vi "waveform-frontpanel.vi"() -> ()   [LabVIEW 2026]
doc: "波形图界面 - 测控软件 多链路实时波形展示。仅前面板布局演示，无程序逻辑。来源：波形图.html 主界面。"
panel:
  out "运行时长":string="运行时长: 00:00:00"
  out "通道":string="通道: 16"
  out "视图":string="视图: 0.0 - 30.0 s"
  out "窗口":string="窗口: 30.0 s"
  out "采样率":string="采样率: 100 Hz / 10 Hz"
  out "链路":string="链路: 4/4 在线"
  out "?":string="滚轮:缩放时间轴 · 左键框选放大 · 右键平移 · 双击复位"
  out "?":string="Δ值 --"
  out "?":string="Δt --"
  out "?":string="C2 --"
  out "?":string="C1 --"
  out "?":string="测量游标未放置 (0/2)"
  out "?":bool
  out "ARINC429 链路":bool=TRUE
  out "CAN 链路":bool=TRUE
  out "OPC 链路":bool=TRUE
  out "TCP 链路":bool=TRUE
  out "可见通道":i32=16
  out "总通道数":i32=23
  out "绘制帧率":string="60 fps"
  out "重绘周期":string="50 ms"
  out "?":string[](array[string])=["\n● 下位机 TCP（100 Hz · 10 通道）\n  ■ 转速 (rpm)\n  ■ 扭矩 (N·m)\n  ■ 排气温度 (℃)\n  ■ 滑油压力 (kPa)\n  ■ 燃油流量 (kg/h)\n  ■ 振动 (g)\n  ■ 进气温度 (℃)\n  ■ 滑油温度 (℃)\n  ■ 启动信号\n  ■ 点火状态\n\n────────────────────────────────\n\n● PLC OPC（10 Hz · 5 通道）\n  ■ 28V 母线电压 (V)\n  ■ 28V 母线电流 (A)\n  ■ 环境温度 (℃)\n  ■ 气源压力 (kPa)\n  ■ 气动阀状态\n\n────────────────────────────────\n\n● CAN 总线（50 Hz · 4 通道）\n  ■ 发电机频率 (Hz)\n  ■ 母线电压 (V)\n  ■ 母线电流 (A)\n  ■ 发电机状态\n\n\n"]
  out "?":waveform(dbl)(graph)
  out "?":string[](array[string])=["\n● 下位机 TCP  ·  在线\n  192.168.1.101:8000\n  PXIC-8840 环形缓冲 · 采样 100 Hz\n  通道 10 个\n\n\n\n\n──────────────────────────────\n\n\n\n\n● PLC OPC  ·  在线\n  opc.tcp://192.168.1.50:4840\n  西门子 S7-1500 · OPC UA · 采样 10 Hz\n  通道 5 个\n\n\n\n\n──────────────────────────────\n\n\n\n\n● CAN 总线  ·  在线\n  CAN1 · 500 kbps\n  PCIe-CAN-2 标准帧 · 采样 50 Hz\n  通道 4 个\n\n\n\n\n──────────────────────────────\n\n\n\n\n● ARINC429  ·  在线\n  429A/L0B1-L0B4\n  PXIe-429-4 4 发 4 收 · 采样 20 Hz\n  通道 4 个\n"]
  in  "通道过滤":i32(ring) items=["全部链路", "仅 TCP", "仅 OPC", "仅 CAN", "仅 ARINC429"]
  in  "Y轴模式":i32(ring) items=["百分比", "物理量程"]
  in  "窗口选择":i32(ring)=30 items=["5 s"=5, "10 s"=10, "15 s"=15, "30 s"=30, "60 s"=60, "120 s"=120]
  in  "清空缓冲":bool
  in  "导出图片":bool
  in  "清除游标":bool
  in  "放置游标":bool
  in  "复位视图":bool
  in  "暂停刷新":bool
  in  "滚动窗口":bool
  out "?":string="--:--:--"
  out "?":string="链路: 4/4 在线"
  out "?":string="● 波形图 | 测控软件 · 多链路实时波形展示"
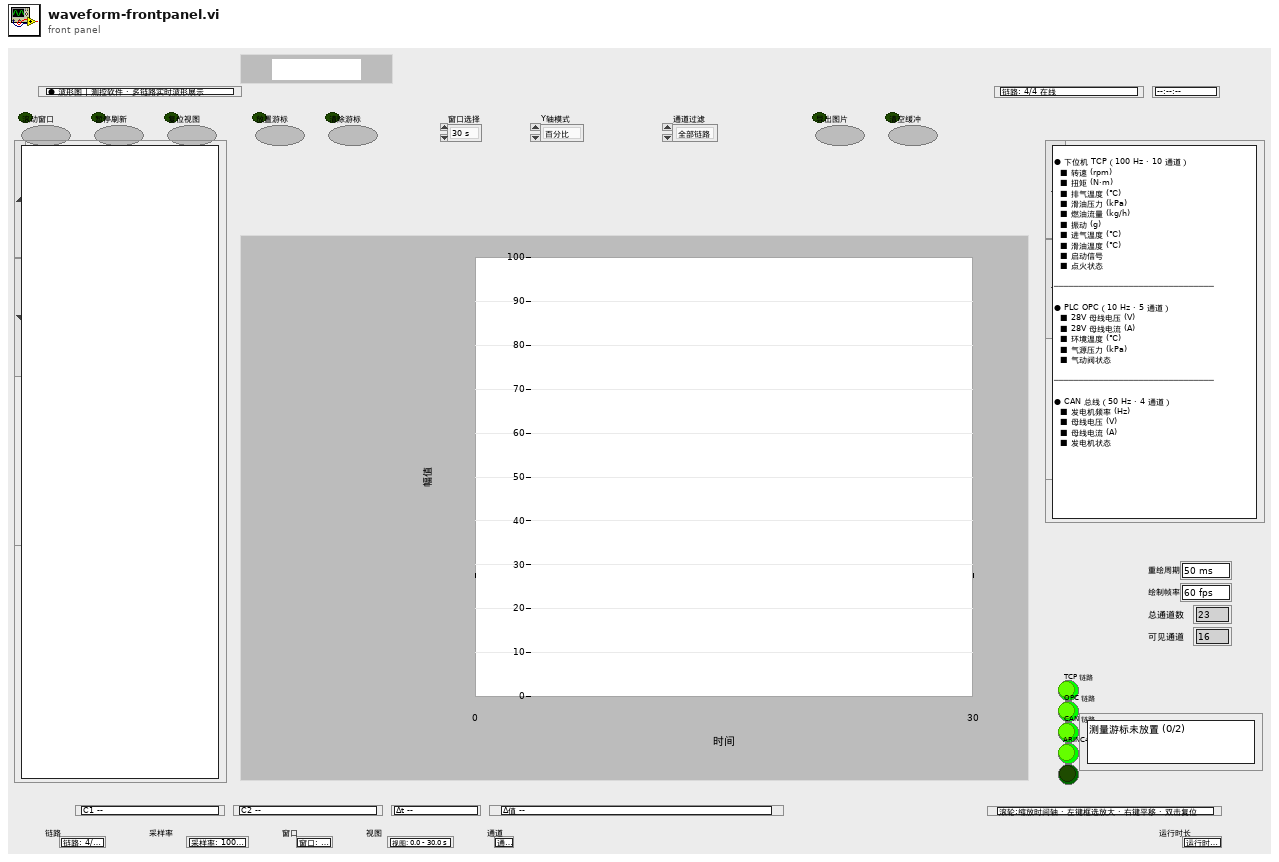
[diagram p1: front panel]
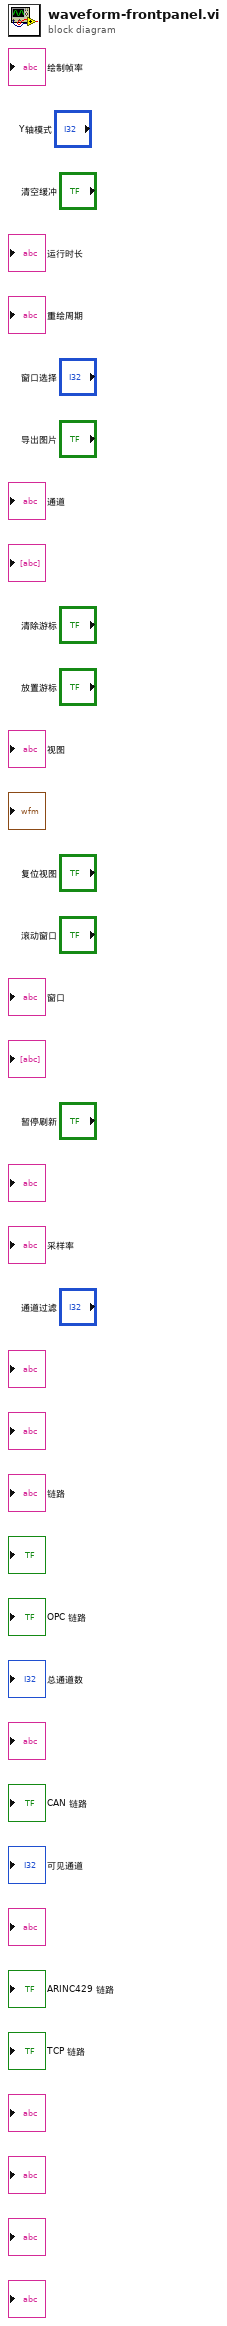
[diagram p0: block diagram]
diagram:
